vi "Pre Launch Init.vi"(11 "DialogBoxSubscribesToDblX in":refnum<class "DialogBoxSubscribesToDblX.lvclass">) -> (0 "error out":errorcluster, 3 "DialogBoxSubscribesToDblX out":refnum<class "DialogBoxSubscribesToDblX.lvclass">)   [LabVIEW 2018, in "DialogBoxSubscribesToDblX.lvclass"]
doc: "(<B>Filename</B>: Actor Framework.lvlib:Actor.lvclass:Pre Launch Init.vi)\n\nDefines behavior that occurs after the Launch Nested Actor method is invoked but before the actor's Actor Core method begins running.\n\nBy default, this method does nothing. A descendant class may override it to define behavior."
uses:
  DialogBoxSubscribesToDblX.lvclass
  Source/IDialogBox/IDialogBox/IDialogBox.lvclass
  cff05223-ea57-43ba-ac96-5a028acbdda5.vi
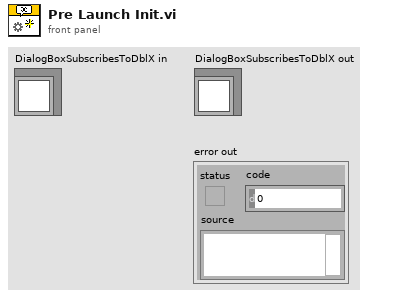
[diagram p1: front panel]
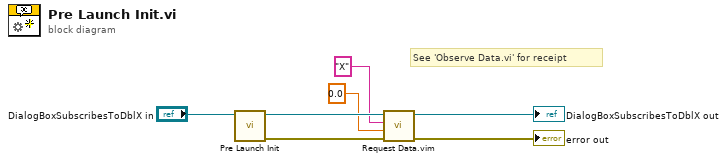
[diagram p0: block diagram]
diagram:
  # "See 'Observe Data.vi' for receipt"
  n1 = call-parent "Pre Launch Init.vi"("IViewable in"="DialogBoxSubscribesToDblX in") -> ("error out"=w7:errorcluster, "IViewable out"=w4:refnum<class "DialogBoxSubscribesToDblX.lvclass">)  [unwired: 9 in]
  n2 = call "Request Data.vim"("error in (no error)"=w7, "Data Type"=0.0, "Datum Name"="X", "IObserver in"=w4) -> ("error out"=→"error out":errorcluster, "IObserver out"=→"DialogBoxSubscribesToDblX out":refnum<class "DialogBoxSubscribesToDblX.lvclass">)  [unwired: 5 in, 1 out]
